vi "SPARK Get Encoder Config.vi"   [LabVIEW 2027]
doc: "Get the configuration of the primary encoder of the SPARK."
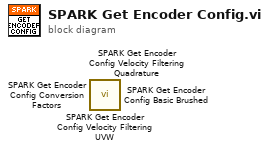
[diagram p0: block diagram]
diagram:
  n1 = call <vilib>:"SPARK Get Encoder Config Velocity Filtering UVW.vi"() -> ()  [unwired: 8 in, 4 out]
  n2 = call <vilib>:"SPARK Get Encoder Config Velocity Filtering Quadrature.vi"() -> ()  [unwired: 8 in, 4 out]
  n3 = call <vilib>:"SPARK Get Encoder Config Conversion Factors.vi"() -> ()  [unwired: 8 in, 4 out]
  n4 = call <vilib>:"SPARK Get Encoder Config Basic Brushed.vi"() -> ()  [unwired: 8 in, 4 out]
